vi "Route Target.vi"(8 "error in (no error)":errorcluster caption="에러 입력(에러 없음)", 10 "Request":string, 11 "Instrument Manager 입력":refnum<class "Instrument Manager.lvclass">) -> (0 "error out":errorcluster caption="에러 출력", 3 "Instrument Manager 출력":refnum<class "Instrument Manager.lvclass">)   [LabVIEW 2023, in "Instrument Manager.lvclass"]
uses:
  Instrument Manager.lvclass
  <vilib>/regexp/Match Regular Expression.xnode
  Instrument Manager.lvclass/Instrument Manager.ctl
panel:
  out "Request 2":string
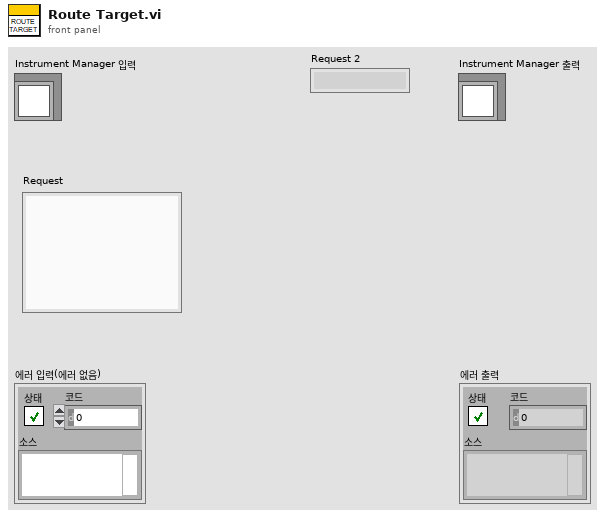
[diagram p1: front panel]
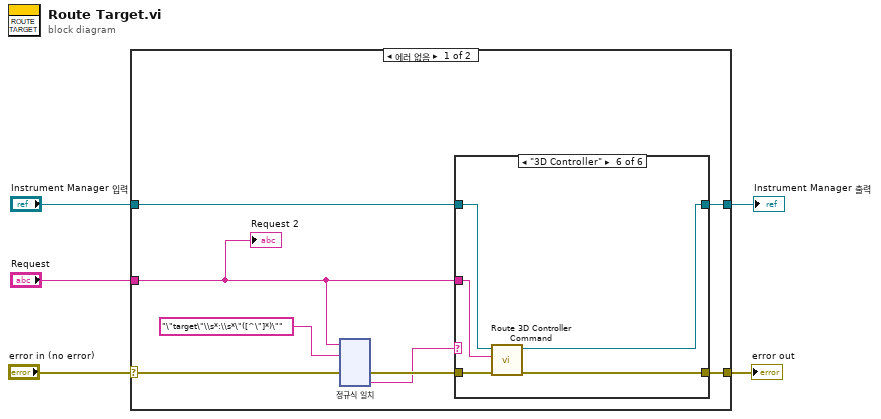
[diagram p0: block diagram]
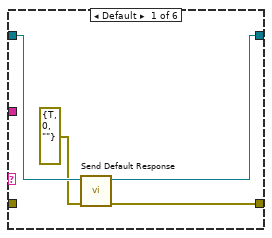
[diagram p2: hidden frame]
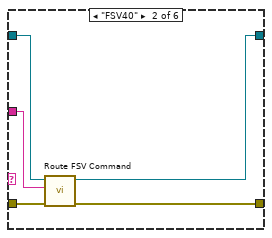
[diagram p3: hidden frame]
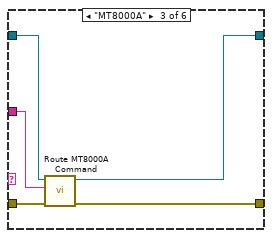
[diagram p4: hidden frame]
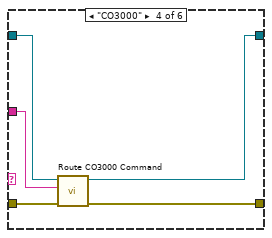
[diagram p5: hidden frame]
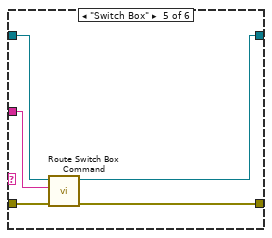
[diagram p6: hidden frame]
diagram:
  n1 = case shown="에러 없음" "error in (no error)" {
    selector: "error in (no error)" -> [w13 w163]
    tunnel: [w10 w163] -> w4
    tunnel: [w7 w162] -> w2
    tunnel: "Instrument Manager 입력" -> [w8 w162]
    tunnel: "Request" -> [w6 _]
    frame No Error {
      n2 = xnode "정규식 일치"("입력 문자열"=w6, "정규식"="\"target\"\\s*:\\s*\"([^\"]*)\"", "에러 입력"=w13) -> ("에러 출력"=w11:errorcluster, "부분 일치 1"=w9:string)  [unwired: 3 in, 4 out]
      n3 = case shown="\"3D Controller\"" w9 {
        tunnel: w11 -> [_ w21 w27 w32 w37 w41]
        tunnel: [w15 w20 w26 w31 w36 w40] -> w10
        tunnel: w8 -> [w17 w22 w24 w30 w35 w39]
        tunnel: [w14 w19 w23 w28 w33 w38] -> w7
        tunnel: w6 -> [_ w18 w25 w29 w34 w42]
        frame Default {
          n4 = call "Send Default Response.vi"("error in (no error)"=errorcluster {"status"=TRUE, "code"=0, "source"=""} ("에러 출력"), "Instrument Manager 입력"=w17) -> ("error out"=w15:errorcluster, "Instrument Manager 출력"=w14:refnum<class "Instrument Manager.lvclass">)  [unwired: 8 in]
        }
        frame "FSV40" {
          n5 = call "Route FSV Command.vi"("error in (no error)"=w21, "문자열"=w18, "Instrument Manager 입력"=w22) -> ("error out"=w20:errorcluster, "Instrument Manager 출력"=w19:refnum<class "Instrument Manager.lvclass">)  [unwired: 7 in]
        }
        frame "MT8000A" {
          n6 = call "Route MT8000A Command.vi"("error in (no error)"=w27, "문자열"=w25, "Instrument Manager 입력"=w24) -> ("error out"=w26:errorcluster, "Instrument Manager 출력"=w23:refnum<class "Instrument Manager.lvclass">)  [unwired: 7 in]
        }
        frame "CO3000" {
          n7 = call "Route CO3000 Command.vi"("error in (no error)"=w32, "문자열"=w29, "Instrument Manager 입력"=w30) -> ("error out"=w31:errorcluster, "Instrument Manager 출력"=w28:refnum<class "Instrument Manager.lvclass">)  [unwired: 7 in]
        }
        frame "Switch Box" {
          n8 = call "Route Switch Box Command.vi"("error in (no error)"=w37, "문자열"=w34, "Instrument Manager 입력"=w35) -> ("error out"=w36:errorcluster, "Instrument Manager 출력"=w33:refnum<class "Instrument Manager.lvclass">)  [unwired: 7 in]
        }
        frame "3D Controller" {
          n9 = call "Route 3D Controller Command.vi"("error in (no error)"=w41, "문자열"=w42, "Instrument Manager 입력"=w39) -> ("error out"=w40:errorcluster, "Instrument Manager 출력"=w38:refnum<class "Instrument Manager.lvclass">)  [unwired: 7 in]
        }
      }
      "Request 2" <- w6
    }
    frame Error {
    }
  }
  "error out" <- w4
  "Instrument Manager 출력" <- w2
